vi "serialization tests.vi"() -> (0 "validation error":errorcluster, 1 "runtime config equal":bool, 2 "config equal":bool, 3 "channels equal":bool, 4 "serialization error":errorcluster)   [LabVIEW 2015, in "E2E Tag Exchange tests.lvlib"]
doc: "Tests the 'To String' and 'From String' methods of the Module's configuration class and ensures they are compatible."
uses:
  E2E Tag Exchange tests.lvlib
  module/configuration/E2E Tag Exchange configuration.lvclass
  module/configuration/Runtime Implementation.ctl
  module/configuration/E2E Tag Exchange configuration.lvclass/E2E Tag Exchange configuration.ctl
  <vilib>/NI/Tag Bus Module Framework/channel/TBM channel.lvclass
  <vilib>/NI/Configuration Framework/serializable configuration/NISE_CEF_serializable configuration.lvclass
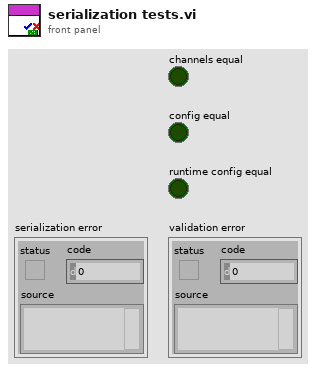
[diagram p1: front panel]
types:
  T1 = typedef "E2E Tag Exchange configuration.lvclass/Runtime Implementation.ctl" = enum16{"RT FIFO", "UDP"}
  T2 = typedef "tag bus.lvlib/tag descriptor.lvclass/Data Type.ctl" = enum16{"Double", "Single", "I64", "I32", "I16", "I8", "U64", "U32", "U16", "U8", "Boolean", "String", "Array of Double", "Array of Single", "Array of I64", "Array of I32", "Array of I16", "Array of I8", "Array of U64", "Array of U32", "Array of U16", "Array of U8", "Array of Boolean", "Array of String"}
  T3 = typedef "TBM channel.lvclass/channel classification.ctl" = enum16{"input data", "output data", "processing parameter", "processing result"}
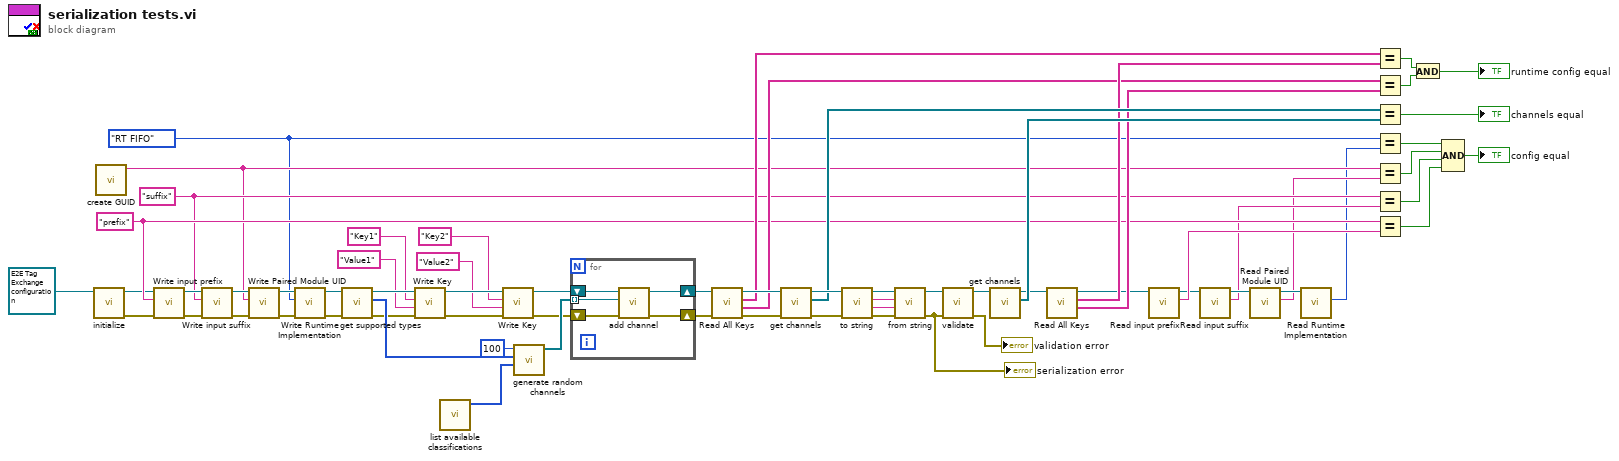
[diagram p0: block diagram]
diagram:
  w10 = Runtime_Implementation."RT FIFO" ("Runtime Implementation")
  w14 = "suffix" ("paired output suffix")
  w18 = "prefix" ("input prefix")
  n1 = call <vilib>:"initialize.vi"("configuration in"=refnum<class "E2E Tag Exchange configuration.lvclass"> refnum ("tag bus configurable plugin module configuration")) -> ("error out"=w2:errorcluster, "configuration out"=w4:refnum<class "E2E Tag Exchange configuration.lvclass">)  [unwired: 8 in, 1 out]
  n2 = call <vilib>:"create GUID.vi"() -> ("uuid"=w12:string)  [unwired: 10 in, 1 out]
  n3 = call "Write input prefix.vi"("error in (no error)"=w2, "input prefix"=w18, "E2E Tag Exchange configuration in"=w4) -> ("error out"=w28:errorcluster, "E2E Tag Exchange configuration out"=w32:refnum<class "E2E Tag Exchange configuration.lvclass">)  [unwired: 7 in]
  n4 = call "Write input suffix.vi"("error in (no error)"=w28, "paired output suffix"=w14, "E2E Tag Exchange configuration in"=w32) -> ("error out"=w29:errorcluster, "E2E Tag Exchange configuration out"=w33:refnum<class "E2E Tag Exchange configuration.lvclass">)  [unwired: 7 in]
  n5 = call "Write Paired Module UID.vi"("error in (no error)"=w29, "Paired Module UID"=w12, "E2E Tag Exchange configuration in"=w33) -> ("error out"=w30:errorcluster, "E2E Tag Exchange configuration out"=w34:refnum<class "E2E Tag Exchange configuration.lvclass">)  [unwired: 7 in]
  n6 = call "Write Runtime Implementation.vi"("error in (no error)"=w30, "Runtime Implementation"=w10, "E2E Tag Exchange configuration in"=w34) -> ("error out"=w31:errorcluster, "E2E Tag Exchange configuration out"=w35:refnum<class "E2E Tag Exchange configuration.lvclass">)  [unwired: 7 in]
  n7 = call-dynamic "get supported types.vi"("error in"=w31, "E2E Tag Exchange configuration in"=w35) -> ("error out"=w27:errorcluster, "supported types"=w36:T2[], "E2E Tag Exchange configuration out"=w38:refnum<class "E2E Tag Exchange configuration.lvclass">)  [unwired: 7 in]
  n8 = call "Write Key.vi"("error in"=w27, "Value"="Value1", "Key"="Key1", "E2E configuration in"=w38) -> ("error out"=w57:errorcluster, "E2E configuration out"=w58:refnum<class "E2E Tag Exchange configuration.lvclass">)  [unwired: 6 in]
  n9 = call <vilib>:"list available classifications.vi"() -> ("supported types"=w37:T3[])  [unwired: 11 in]
  n10 = call "Write Key.vi"("error in"=w57, "Value"="Value2", "Key"="Key2", "E2E configuration in"=w58) -> ("error out"=w59:errorcluster, "E2E configuration out"=w60:refnum<class "E2E Tag Exchange configuration.lvclass">)  [unwired: 6 in]
  n11 = call "generate random channels.vi"("Supported Channel Classifications"=w37, "supported types"=w36, "Number of Random Channels to Create"=100) -> ("Random Channels"=w66:refnum<class "TBM channel.lvclass">[])  [unwired: 8 in]
  n12 = for {
    shift-right: [w70] -> w56
    shift-left: w60 -> [w71]
    tunnel: w66 -> [w69] mode=indexing
    shift-right: [w67] -> w54
    shift-left: w59 -> [w68]
    n13 = call "add channel.vi"("error in (no error)"=w68, "channel"=w69, "E2E configuration in"=w71) -> ("error out"=w67:errorcluster, "E2E configuration out"=w70:refnum<class "E2E Tag Exchange configuration.lvclass">)  [unwired: 7 in]
  }
  n14 = call "Read All Keys.vi"("error in"=w54, "E2E configuration in"=w56) -> ("error out"=w53:errorcluster, "Values"=w47:string[], "Keys"=w50:string[], "E2E configuration out"=w55:refnum<class "E2E Tag Exchange configuration.lvclass">)  [unwired: 6 in]
  n15 = call-dynamic "get channels.vi"("E2E configuration in"=w55) -> ("channels"=w51:refnum<class "TBM channel.lvclass">[], "E2E configuration out"=w63:refnum<class "E2E Tag Exchange configuration.lvclass">)  [unwired: 9 in]
  n16 = call-dynamic "to string.vi"("error in"=w53, "E2E Tag Exchange configuration in"=w63) -> ("error out"=w64:errorcluster, "data"=w61:string, "version"=w62:string, "E2E Tag Exchange configuration out"=w65:refnum<class "E2E Tag Exchange configuration.lvclass">)  [unwired: 6 in]
  n17 = call-dynamic "from string.vi"("error in"=w64, "data"=w61, "version"=w62, "E2E Tag Exchange configuration in"=w65) -> ("error out"=w40:errorcluster, "E2E Tag Exchange configuration out"=w43:refnum<class "E2E Tag Exchange configuration.lvclass">)  [unwired: 6 in]
  "serialization error" <- w40
  n18 = call-dynamic "validate.vi"("error in"=w40, "E2E Tag Exchange configuration in"=w43) -> ("error out"=→"validation error":errorcluster, "E2E Tag Exchange configuration out"=w42:refnum<class "E2E Tag Exchange configuration.lvclass">)  [unwired: 8 in]
  n19 = call-dynamic "get channels.vi"("E2E configuration in"=w42) -> ("channels"=w52:refnum<class "TBM channel.lvclass">[], "E2E configuration out"=w49:refnum<class "E2E Tag Exchange configuration.lvclass">)  [unwired: 9 in]
  n20 = call "Read All Keys.vi"("E2E configuration in"=w49) -> ("Values"=w46:string[], "Keys"=w48:string[], "E2E configuration out"=w22:refnum<class "E2E Tag Exchange configuration.lvclass">)  [unwired: 7 in, 1 out]
  n21 = call "Read input prefix.vi"("E2E Tag Exchange configuration in"=w22) -> ("input prefix"=w19:string, "E2E Tag Exchange configuration out"=w17:refnum<class "E2E Tag Exchange configuration.lvclass">)  [unwired: 8 in, 1 out]
  n22 = call "Read input suffix.vi"("E2E Tag Exchange configuration in"=w17) -> ("input suffix"=w15:string, "E2E Tag Exchange configuration out"=w16:refnum<class "E2E Tag Exchange configuration.lvclass">)  [unwired: 8 in, 1 out]
  n23 = call "Read Paired Module UID.vi"("E2E Tag Exchange configuration in"=w16) -> ("Paired Module UID"=w13:string, "E2E Tag Exchange configuration out"=w21:refnum<class "E2E Tag Exchange configuration.lvclass">)  [unwired: 8 in, 1 out]
  n24 = call "Read Runtime Implementation.vi"("E2E Tag Exchange configuration in"=w21) -> ("Runtime Implementation"=w11:T1)  [unwired: 8 in, 2 out]
  n25 = Equal?(x=w50, y=w48) -> (x = y?=w45:bool)
  n26 = Equal?(x=w47, y=w46) -> (x = y?=w44:bool)
  n27 = Equal?(x=w51, y=w52) -> (x = y?=→"channels equal":bool)
  n28 = Equal?(x=w10, y=w11) -> (x = y?=w9:bool)
  n29 = Equal?(x=w12, y=w13) -> (x = y?=w8:bool)
  n30 = Equal?(x=w14, y=w15) -> (x = y?=w7:bool)
  n31 = Equal?(x=w18, y=w19) -> (x = y?=w6:bool)
  n32 = And(x=w45, y=w44) -> (x .and. y?=→"runtime config equal":bool)
  n33 = Compound Arithmetic op=AND(w9, w8, w7, w6) -> (→"config equal":bool)
